vi "Reject Invalid Request.vi"(8 "error in":errorcluster, 10 "response":string, 11 "request":string) -> (0 "error out":errorcluster, 3 "response out":string)   [LabVIEW 2020, in "MCP Server.lvlib"]
doc: "A message that is a valid JSON object but has no method is not a request: the answer is JSON-RPC error -32600 (Invalid Request). Restore Request ID.vi puts the id of the message in afterwards.\n\nA message that is valid JSON but not an object gets the same error from Reject Non Object Message.vi. Every other response is passed through, so an empty or unparsable body keeps its -32700 (Parse error) answer."
uses:
  MCP Server.lvlib
  <vilib>/JDP Science/JSONtext/Next JSON Value.vi
  <vilib>/JDP Science/JSONtext/String Subset.vi
  <vilib>/JDP Science/JSONtext/Parsing/Advance past next JSON Value (inlined COPY).vi
  <vilib>/JDP Science/JSONtext/Parsing/Advance past whitespace.vi
  <vilib>/JDP Science/JSONtext/Parsing/Advance past String.vi
  <vilib>/JDP Science/JSONtext/Parsing/Advance past Number.vi
  <vilib>/JDP Science/JSONtext/Parsing/Advance past Line Ending.vi
  <vilib>/JDP Science/JSONtext/Parsing/Parse Full Path or Item Name.vi
  <vilib>/JDP Science/JSONtext/Parsing/Advance past Array.vi
  <vilib>/JDP Science/JSONtext/Parsing/Advance past Object.vi
  <vilib>/JDP Science/JSONtext/support/Error Cluster From Code.vi
  <vilib>/JDP Science/JSONtext/Offset/Find Item Locations by Path.vi
  <vilib>/JDP Science/JSONtext/JSONtext.lvlib
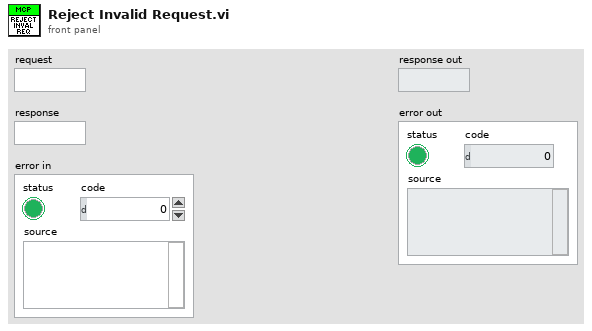
[diagram p1: front panel]
types:
  T1 = typedef "JSONtext.lvlib/JSON Value Type.ctl" = enum16{"Not a JSON Value", "JSON Object", "JSON Array", "String", "Number", "true", "false", "null"}
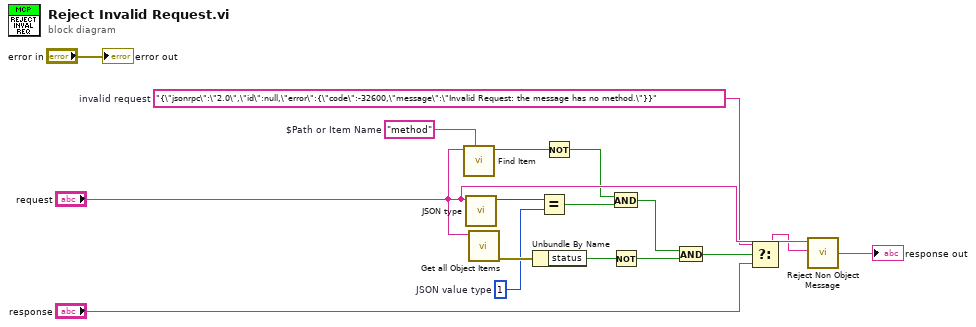
[diagram p0: block diagram]
diagram:
  w6 = "{\"jsonrpc\":\"2.0\",\"id\":null,\"error\":{\"code\":-32600,\"message\":\"Invalid Request: the message has no method.\"}}"  # invalid request
  w12 = u16 1  # JSON value type
  w17 = "method"  # $Path or Item Name
  n1 = call <vilib>:"Find Item.vi"("$Path or Item Name"=w17, "JSON"="request") -> ("Found"=w15:bool)  [unwired: 6 in, 3 out]
  n2 = call <vilib>:"JSON type.vi"("JSON"="request") -> ("JSON Value Type"=w13:T1)  [unwired: 9 in, 1 out]
  n3 = call <vilib>:"Get all Object Items.vi"("JSON"="request") -> ("error out"=w16:errorcluster)  [unwired: 7 in, 3 out]
  n4 = Unbundle By Name(w16) -> ("status"=w11:bool)
  n5 = Equal?(x=w13, y=w12) -> (x = y?=w9:bool)
  n6 = Not(x=w15) -> (.not. x?=w10:bool)
  n7 = And(x=w10, y=w9) -> (x .and. y?=w8:bool)
  n8 = Not(x=w11) -> (.not. x?=w7:bool)
  n9 = And(x=w8, y=w7) -> (x .and. y?=w5:bool)
  n10 = Select(t=w6, s=w5, f="response") -> (s? t:f=w1:string)
  n11 = call "Reject Non Object Message.vi"("response"=w1, "request"="request") -> ("response out"=→"response out":string)  [unwired: 8 in, 1 out]
  "error out" <- "error in"
